vi "test--Black.vi"(11 "Test Case In":refnum<class "Color to HSL.lvclass">) -> (0 "error out":errorcluster, 3 "Test Case Out":refnum<class "Color to HSL.lvclass">)   [LabVIEW 2021, in "Color to HSL.lvclass"]
uses:
  Color to HSL.lvclass
  C:/Program Files/National Instruments/LabVIEW 2024/vi.lib/Astemes/LUnit/Test Case.lvclass
  <vilib>/Astemes/LUnit/Test Case.lvclass/Test Case.ctl
  4993e8ee-a06a-463a-9684-69129f64d5ce.vi
  e1f6035f-84b0-47d9-b4e6-4c80e5700516.vi
  65188c90-562b-40a8-ad2d-cbd4f2c1f132.vi
  <vilib>/Astemes/LUnit/Core/LUnit Test Case/Private/Append Pass Result.vi
  <vilib>/Astemes/LUnit/Core/LUnit Test Case/Private/Append Fail Result.vi
  4993e8ee-a06a-463a-9684-69129f64d5ce.vi/9c5d11cd-9439-4240-a1ee-d9baace9c924.vi
  e1f6035f-84b0-47d9-b4e6-4c80e5700516.vi/9c5d11cd-9439-4240-a1ee-d9baace9c924.vi
  65188c90-562b-40a8-ad2d-cbd4f2c1f132.vi/9c5d11cd-9439-4240-a1ee-d9baace9c924.vi
  <vilib>/Astemes/LUnit/Core/LUnit Test Case/Private/Run In UI.vi
  <vilib>/Utility/error.llb/Clear Errors.vi
  <vilib>/Utility/colorconv.llb/Color to RGB.vi
  src/Material SubVIs/Material SubVIs.lvlib
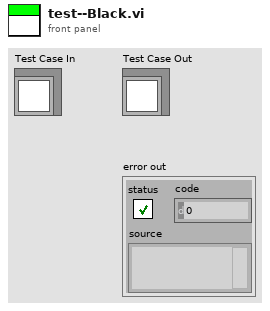
[diagram p1: front panel]
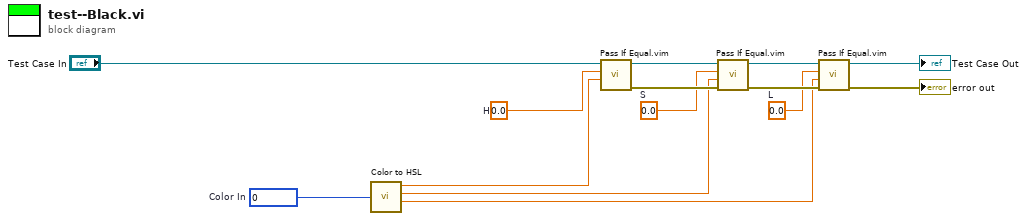
[diagram p0: block diagram]
diagram:
  w2 = 0.0  # L
  w3 = 0.0  # S
  w11 = 0.0  # H
  w13 = u32 0  # Color In
  n1 = call "Color to HSL.vi"("Color In"=w13) -> ("H (degrees)"=w12:dbl, "S (%)"=w4:dbl, "L (%)"=w1:dbl)  [unwired: 4 in, 1 out]
  n2 = call "Pass If Equal.vim"("Actual"=w12, "Expected"=w11, "LUnit Test Case In"="Test Case In") -> ("error out"=w5:errorcluster, "LUnit Test Case Out"=w10:refnum<class "Color to HSL.lvclass">)  [unwired: 7 in]
  n3 = call "Pass If Equal.vim"("error in (no error)"=w5, "Actual"=w4, "Expected"=w3, "LUnit Test Case In"=w10) -> ("error out"=w6:errorcluster, "LUnit Test Case Out"=w8:refnum<class "Color to HSL.lvclass">)  [unwired: 6 in]
  n4 = call "Pass If Equal.vim"("error in (no error)"=w6, "Actual"=w1, "Expected"=w2, "LUnit Test Case In"=w8) -> ("error out"=→"error out":errorcluster, "LUnit Test Case Out"=→"Test Case Out":refnum<class "Color to HSL.lvclass">)  [unwired: 6 in]
